vi "ReadConfigToControl.vi"(7 "VI引用句柄":refnum<vi>, 8 "error in (no error)":errorcluster caption="错误输入（无错误）", 9 "ConfigInfo":T1(array[cluster]), 10 "section":string caption="段", 11 "refnum":refnum<k1>) -> (0 "error out":errorcluster caption="错误输出", 3 "refnum out":refnum<k1> caption="refnum")   [LabVIEW 2025]
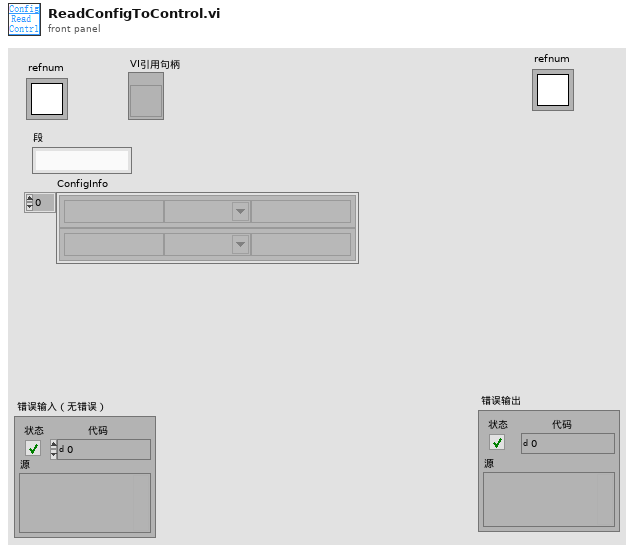
[diagram p1: front panel]
types:
  T1 = cluster{"Name":string, "Type":string, "DefVal":string}[]
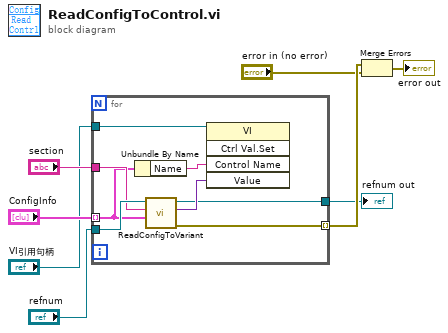
[diagram p0: block diagram]
diagram:
  n1 = for {
    tunnel: "ConfigInfo" -> [w13] mode=indexing
    tunnel: "section" -> [w14]
    tunnel: "refnum" -> [w15]
    tunnel: [w11] -> w5 mode=indexing
    tunnel: [w9] -> w2
    tunnel: "VI引用句柄" -> [w10]
    n2 = Unbundle By Name(w13) -> ("Name"=w16:string)
    n3 = call "ReadConfigToVariant.vi"("Info"=w13, "section"=w14, "Configrefnum"=w15) -> ("error out"=w11:errorcluster, "Variant"=w12:variant, "Configrefnum out"=w9:refnum<k1>)  [unwired: 6 in]
    n4 = invoke class="VI" method="Ctrl Val.Set"(reference=w10, "Control Name"=w16, "Value"=w12) -> ()  [unwired: 2 in, 5 out]
  }
  "refnum out" <- w2
  n5 = Merge Errors(w5, "error in (no error)") -> (→"error out":errorcluster)
